vi "ADC.vi"(0 "Instrument Handle In":refnum<k15>, 1 "ADC Resolution":u32, 5 "Start Voltage":dbl, 7 "Stop Voltage":dbl, 9 "Step Size":dbl, 11 "Error In":errorcluster, 12 "ADC Full Scale Voltage":dbl) -> (4 "Instrument Handle Out":refnum<k15>, 6 "Voltage":dbl[](array[numeric]), 8 "Code":i32[](array[numeric]), 15 "Error Out":errorcluster)   [LabVIEW 2026, in "Core.lvlib"]
doc: "This VI acts as an ADC."
uses:
  Core.lvlib
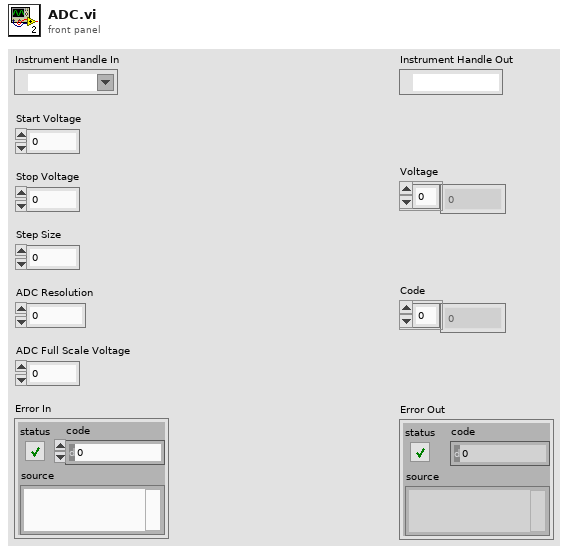
[diagram p1: front panel]
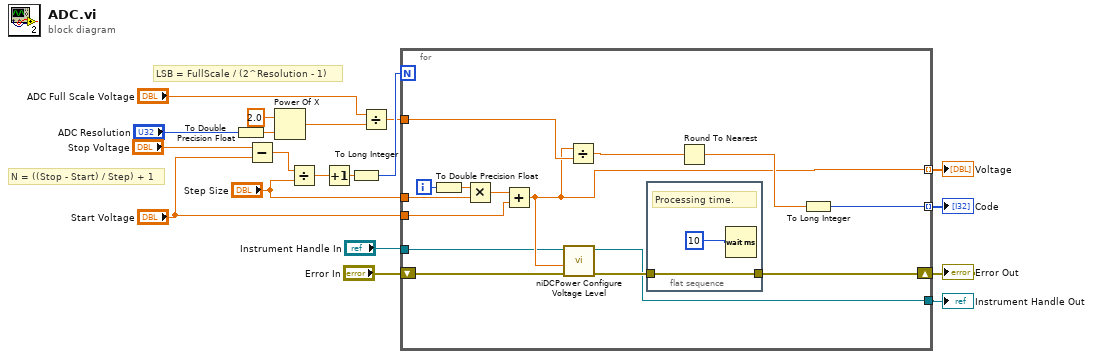
[diagram p0: block diagram]
diagram:
  # "LSB = FullScale / (2^Resolution - 1)"
  # "N = ((Stop - Start) / Step) + 1"
  n1 = To Double Precision Float(number="ADC Resolution") -> (double precision float=w7:dbl)
  n2 = Subtract(x="Stop Voltage", y="Start Voltage") -> (x-y=w18:dbl)
  n3 = Power Of X(1:w7, 2:2.0 ("y")) -> (0:w6:dbl)
  n4 = Divide(x=w18, y="Step Size") -> (x/y=w17:dbl)
  n5 = Increment(x=w17) -> (x+1=w16:dbl)
  n6 = To Long Integer(number=w16) -> (32bit integer=w15:i32)
  n7 = Divide(x="ADC Full Scale Voltage", y=w6) -> (x/y=w5:dbl)
  n8 = for {
    N: w15 -> [_]
    tunnel: "Step Size" -> [w34]
    tunnel: "Start Voltage" -> [w30]
    shift-right: [w27] -> w1
    shift-left: "Error In" -> [w29]
    tunnel: [w22] -> w12 mode=indexing
    tunnel: [w23] -> w11 mode=indexing
    tunnel: w5 -> [w26]
    tunnel: "Instrument Handle In" -> [w21]
    tunnel: [w20] -> w3
    i -> [w33]
    n9 = To Double Precision Float(number=w33) -> (double precision float=w32:dbl)
    n10 = Multiply(x=w32, y=w34) -> (x*y=w31:dbl)
    n11 = Add(x=w31, y=w30) -> (x+y=w22:dbl)
    n12 = call <instrlib>:"niDCPower Configure Voltage Level.vi"("error in (no error)"=w29, "voltage level"=w22, "instrument handle"=w21) -> ("error out"=w28:errorcluster, "instrument handle out"=w20:refnum<k15>)  [unwired: 7 in]
    n13 = Divide(x=w22, y=w26) -> (x/y=w25:dbl)
    n14 = flat-sequence {
      tunnel: w28 -> [w35]
      tunnel: [w35] -> w27
      frame #0 {
        # "Processing time."
        n15 = Wait (ms)(milliseconds to wait=u32 10) -> ()  [unwired: 1 out]
      }
    }
    n16 = Round To Nearest(number=w25) -> (nearest integer value=w24:dbl)
    n17 = To Long Integer(number=w24) -> (32bit integer=w23:i32)
  }
  "Voltage" <- w12
  "Code" <- w11
  "Instrument Handle Out" <- w3
  "Error Out" <- w1
